vi "Assert True.vi"(8 "error in":errorcluster, 10 "failure message":string, 11 "condition":bool) -> (0 "error out":errorcluster, 2 "message":string, 3 "pass":bool)   [LabVIEW 2021, in "MeasurementServerTests.lvlib"]
uses:
  MeasurementServerTests.lvlib
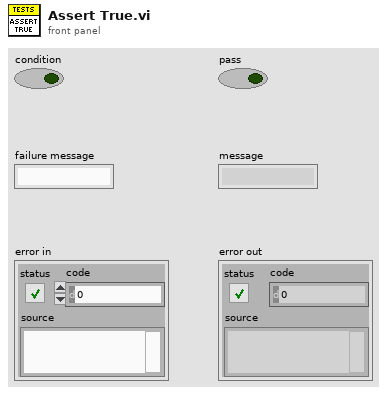
[diagram p1: front panel]
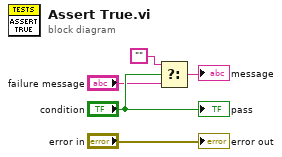
[diagram p0: block diagram]
diagram:
  n1 = Select(t="", s="condition", f="failure message") -> (s? t:f=→"message":string)
  "error out" <- "error in"
  "pass" <- "condition"
